vi "Transmitter_Example_V4.vi"() -> ()   [LabVIEW 2022 SP3]
uses:
  <instrlib>/niUSRP/niUSRP Write Tx Data (CDB Cluster).vi
panel:
  out "Numeric":i32
  in  "Frames":i32=5000
  in  "Timer":bool
  in  "Modulation parameter LP":T1
  in  "String Critical Data 2":string="Critical Dataaaaa\nCritical Dataaaaa\nCritical Dataaaaa\nCritical Dataaaaa\nCritical Dataaaaa\nNon Critical Data\nNon Critical Data\nNon Critical Data\nNon Critical Data\nNon Critical Data"
  in  "milliseconds to wait":u32=100
  in  "OFDM 4QAM / 16QAM":bool
  out "AuxString 2":string
  out "AuxString":string
  in  "Previous Button":bool caption="Both Critical and Non Critical\nData must be equal size."
  in  "New Critical Data":string="Non Critical Data\nNon Critical Data\nNon Critical Data\nNon Critical Data\nNon Critical Data"
  in  "New Non Critical Data":string="Critical Dataaaaa\nCritical Dataaaaa\nCritical Dataaaaa\nCritical Dataaaaa\nCritical Dataaaaa"
  out "Frame Duration 2":dbl format="%#_6p"
  in  "Alpha":dbl=0.05 min=0.0 max=1.0 step=0.05
  out "Bits length 2":i32
  in  "String Critical Data":string="Non Critical Data\nNon Critical Data\nNon Critical Data\nNon Critical Data\nNon Critical Data\n"
  in  "Modulation parameter HP":T1
  out "Bits length":i32
  out "Frame Duration":dbl format="%#_6p"
  out "Waveform Graph":cluster{"t0":dbl, "dt":dbl, "Y":dbl[]}(graph)
  in  "stop":bool
  in  "String Non Critical Data":string="Critical Dataaaaa\nCritical Dataaaaa\nCritical Dataaaaa\nCritical Dataaaaa\nCritical Dataaaaa\n"
  out "USRP CoercedParamters":T2={"coerced IQ rate"=100000.0, "coerced carrier frequency"=100000.0, "coerced gain"=0.0} {"coerced gain" format="%#_6f"; "coerced carrier frequency" format="%#_6p"; "coerced IQ rate" format="%#_6p"}
  out "error out":errorcluster
  in  "error in (no error)":errorcluster
  in  "USRP ControledParameters":T3={"active antenna"="TX1", "gain"=20.0, "carrier frequency"=2400000000.0, "IQ rate"=2000000.0} {"IQ rate" format="%#_6p"; "carrier frequency" format="%#_6p"; "gain" format="%#_6f"}
  in  "device names":refnum<k15>="RIO0"
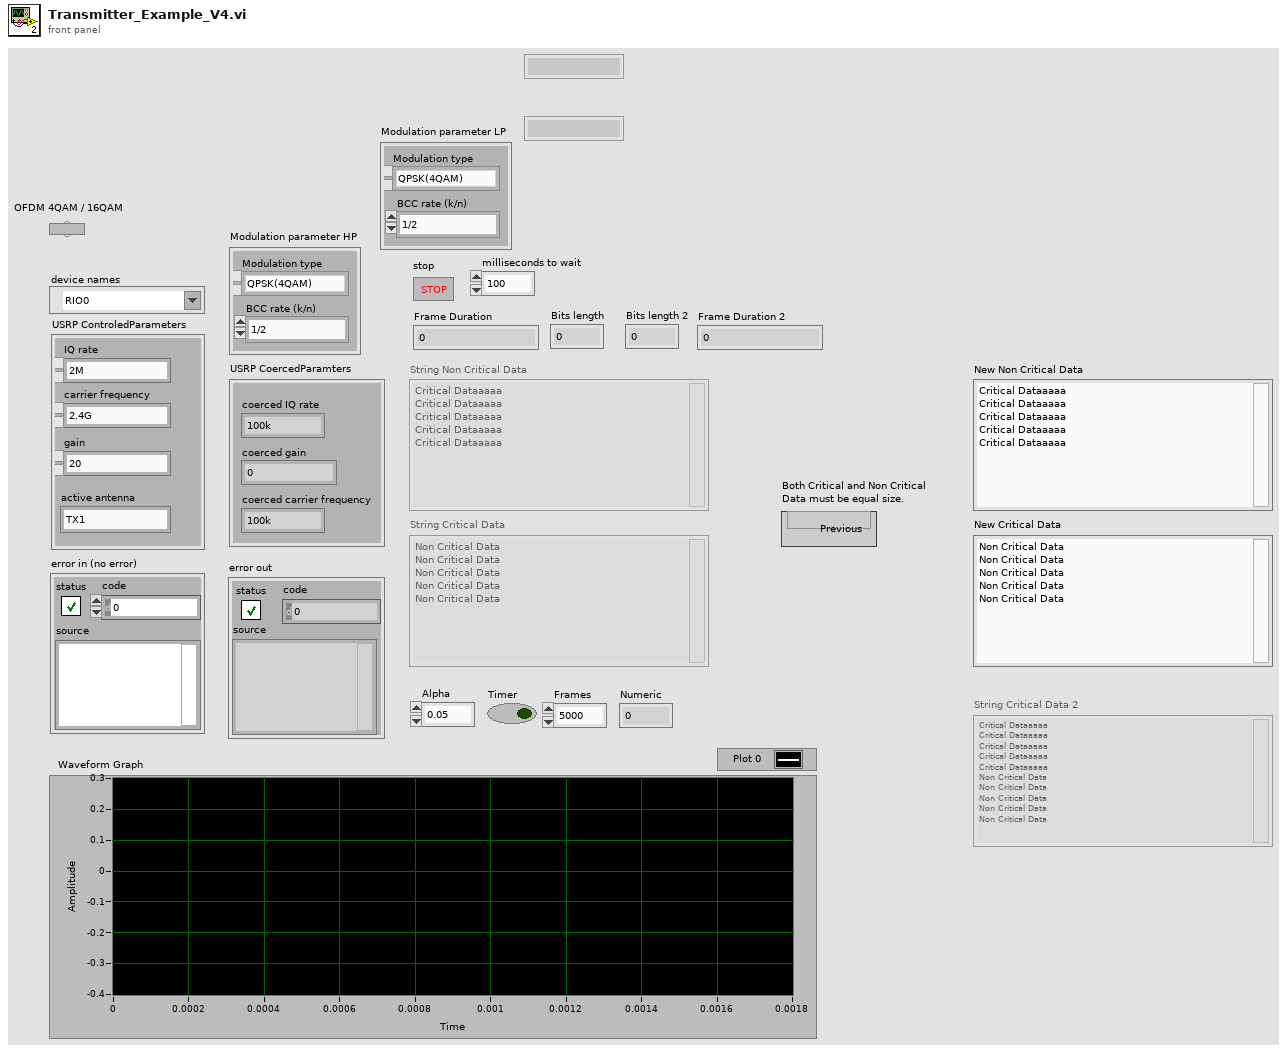
[diagram p1: front panel]
types:
  T1 = cluster{"Modulation type":enum16{"QPSK(4QAM)", "64QAM", "16QAM", "BPSK"}, "BCC rate (k/n)":enum16{"1/2", "2/3", "3/4"}}
  T2 = cluster{"coerced IQ rate":dbl, "coerced carrier frequency":dbl, "coerced gain":dbl}
  T3 = cluster{"active antenna":string, "gain":dbl, "carrier frequency":dbl, "IQ rate":dbl}
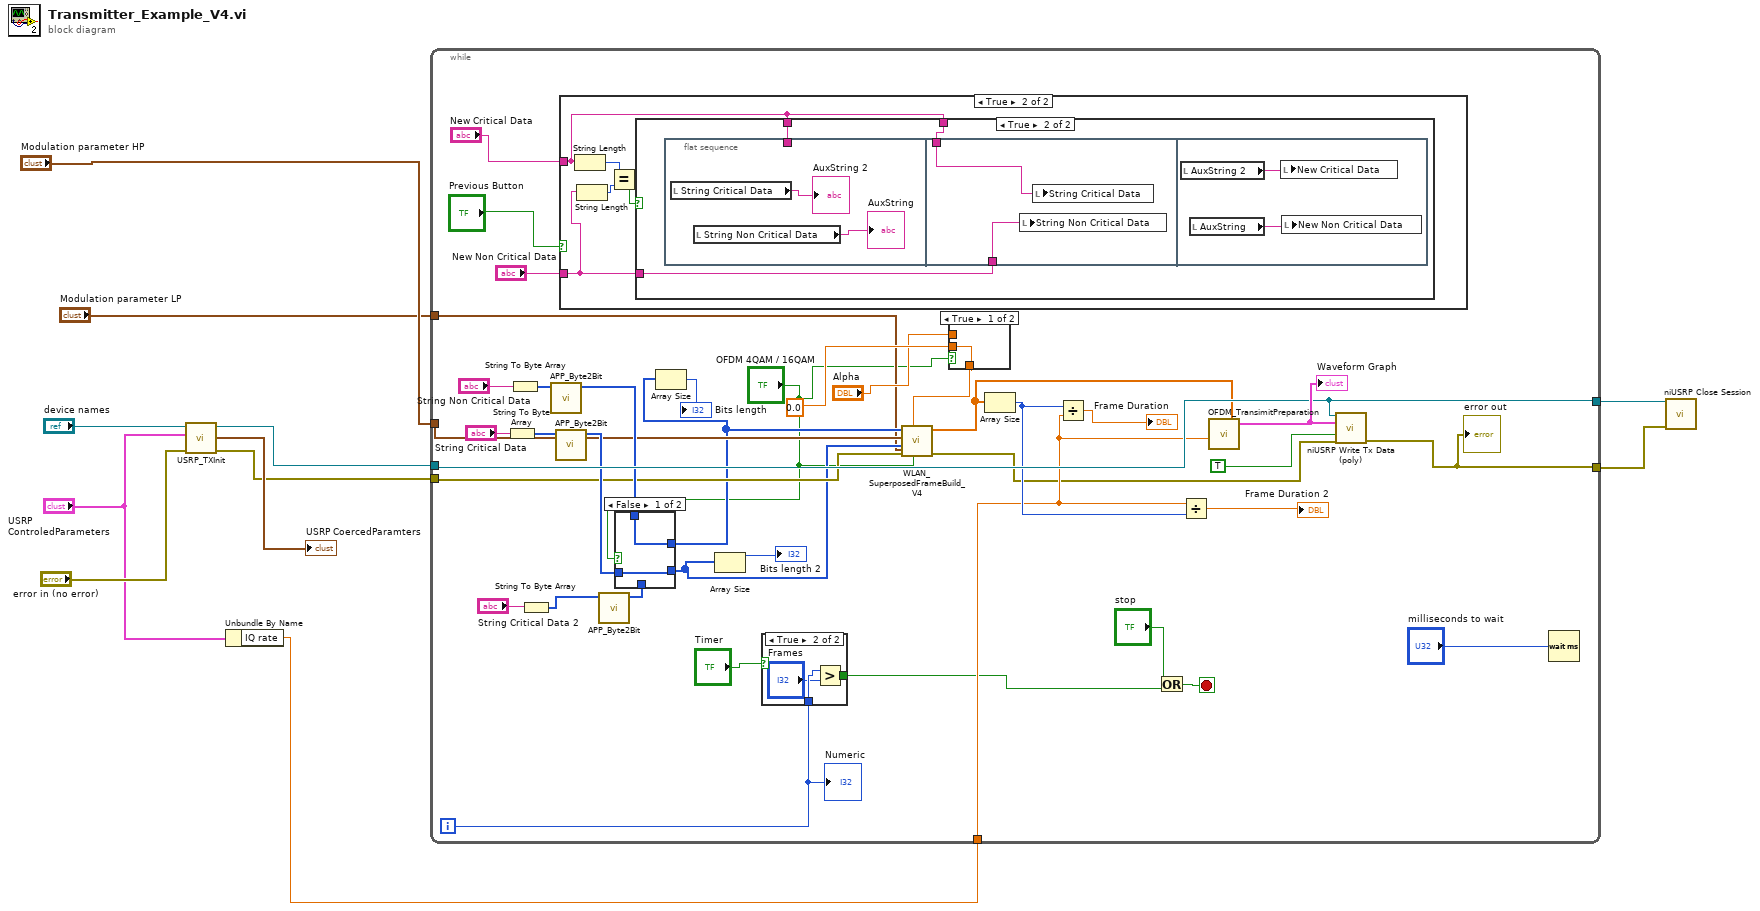
[diagram p0: block diagram]
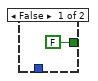
[diagram p2: hidden frame]
diagram:
  n1 = call "USRP_TXInit.vi"("device names"="device names", "USRP ControledParameters"="USRP ControledParameters", "error in (no error)"="error in (no error)") -> ("session handle out"=w9:refnum<k15>, "USRP CoercedParamters"=→"USRP CoercedParamters":T2, "error out"=w6:errorcluster)  [unwired: 5 in]
  n2 = Unbundle By Name("USRP ControledParameters") -> ("IQ rate"=w3:dbl)
  n3 = while {
    tunnel: w9 -> [w46]
    tunnel: "Modulation parameter HP" -> [w22]
    tunnel: w6 -> [w24]
    tunnel: w3 -> [w40]
    tunnel: [w46] -> w5
    tunnel: [w45] -> w4
    tunnel: "Modulation parameter LP" -> [w18]
    i -> [w14]
    stop <- w15 stop-if-true
    n4 = String To Byte Array(string="String Critical Data") -> (unsigned byte array=w42:u8[])
    n5 = String To Byte Array(string="String Non Critical Data") -> (unsigned byte array=w43:u8[])
    n6 = String To Byte Array(string="String Critical Data 2") -> (unsigned byte array=w30:u8[])
    n7 = call "APP_Byte2Bit.vi"("input byte stream"=w43) -> ("output bit stream"=w27:i8[])  [unwired: 10 in]
    n8 = call "APP_Byte2Bit.vi"("input byte stream"=w42) -> ("output bit stream"=w29:i8[])  [unwired: 10 in]
    n9 = case shown="True" "Previous Button" {
      tunnel: "New Non Critical Data" -> [_ w64]
      tunnel: "New Critical Data" -> [_ w60]
      frame False {
      }
      frame True {
        n10 = String Length(string=w60) -> (length=w63:i32)
        n11 = String Length(string=w64) -> (length=w62:i32)
        n12 = Equal?(x=w63, y=w62) -> (x = y?=w61:bool)
        n13 = case shown="True" w61 {
          tunnel: w64 -> [_ w67]
          tunnel: w60 -> [_ w66]
          tunnel: w60 -> [_ w65]
          frame False {
          }
          frame True {
            n14 = flat-sequence {
              tunnel: w65 -> [_]
              tunnel: w67 -> [w71]
              tunnel: w66 -> [w70]
              frame #0 {
                n15 = local read "String Critical Data"() -> (→"AuxString 2":string)
                n16 = local read "String Non Critical Data"() -> (→"AuxString":string)
              }
              frame #1 {
                n17 = local write "String Non Critical Data"(w71) -> ()
                n18 = local write "String Critical Data"(w70) -> ()
              }
              frame #2 {
                n19 = local read "AuxString 2"() -> (w72:string)
                n20 = local read "AuxString"() -> (w73:string)
                n21 = local write "New Critical Data"(w72) -> ()
                n22 = local write "New Non Critical Data"(w73) -> ()
              }
            }
          }
        }
      }
    }
    n23 = call "APP_Byte2Bit.vi"("input byte stream"=w30) -> ("output bit stream"=w28:i8[])  [unwired: 10 in]
    n24 = case shown="False" "OFDM 4QAM / 16QAM" {
      tunnel: [w56 w57] -> w23
      tunnel: w29 -> [w56 _]
      tunnel: w28 -> [_ w57]
      tunnel: [w55 w57] -> w21
      tunnel: w27 -> [w55 _]
      frame False {
      }
      frame True {
      }
    }
    n25 = Array Size(array=w21) -> (size(s)=→"Bits length":i32)
    n26 = Array Size(array=w23) -> (size(s)=→"Bits length 2":i32)
    n27 = case shown="True" "Timer" {
      tunnel: w14 -> [_ w54]
      tunnel: [FALSE w53] -> w13
      frame False {
      }
      frame True {
        n28 = Greater?(x=w54, y="Frames") -> (0:w53:bool)
      }
    }
    n29 = case shown="True" "OFDM 4QAM / 16QAM" {
      tunnel: [w58 w59] -> w20
      tunnel: "Alpha" -> [_ w59]
      tunnel: 0.0 ("Alpha 2") -> [w58 _]
      frame True {
      }
      frame False {
      }
    }
    n30 = call "WLAN_SuperposedFrameBuild_V4.vi"("Modulation parameter LP"=w18, "OFDMON"="OFDM 4QAM / 16QAM", "Alpha"=w20, "error in (no error)"=w24, "data in 2"=w23, "Modulation parameter HP"=w22, "data in"=w21) -> ("error out"=w25:errorcluster, "output array"=w19:cdb[])  [unwired: 3 in]
    n31 = Array Size(array=w19) -> (size(s)=w41:i32)
    n32 = Divide(x=w41, y=w40) -> (x/y=→"Frame Duration":dbl)
    n33 = Or(x="stop", y=w13) -> (x .or. y?=w15:bool)
    n34 = Divide(x=w40, y=w41) -> (x/y=→"Frame Duration 2":dbl)
    n35 = call "OFDM_TransimitPreparation.vi"("IQ rate"=w40, "array"=w19) -> ("output cluster"=w48:cluster{"t0":dbl, "dt":dbl, "Y":cdb[]})  [unwired: 9 in]
    "Waveform Graph" <- w48
    n36 = call-poly <instrlib>:"niUSRP Write Tx Data (poly).vi"("session handle"=w46, "data"=w48, "end of data?"=TRUE, "error in (no error)"=w25) -> ("error out"=w45:errorcluster)  [unwired: 10 in, 1 out]
    "error out" <- w45
    n37 = Wait (ms)(milliseconds to wait="milliseconds to wait") -> ()  [unwired: 1 out]
    "Numeric" <- w14
  }
  n38 = call <instrlib>:"niUSRP Close Session.vi"("session handle"=w5, "error in (no error)"=w4) -> ()  [unwired: 13 in, 1 out]
